vi "move folder contents up one hierarchy level.vi"(10 "error in":errorcluster, 11 "file":path) -> (2 "error out":errorcluster)   [LabVIEW 2014]
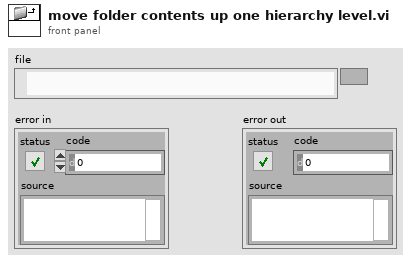
[diagram p1: front panel]
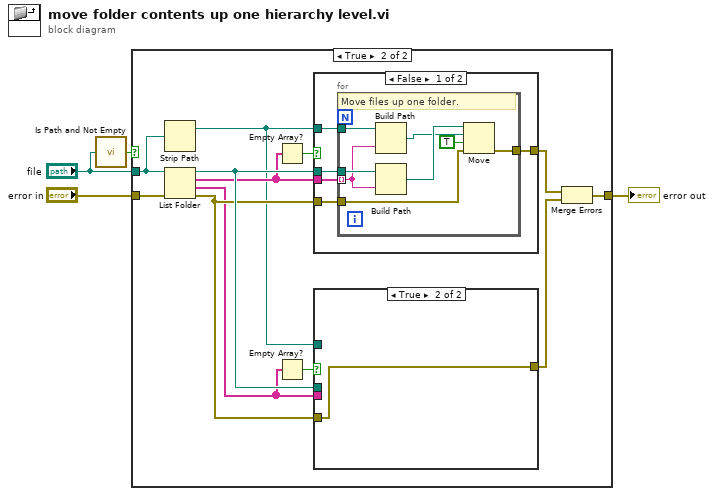
[diagram p0: block diagram]
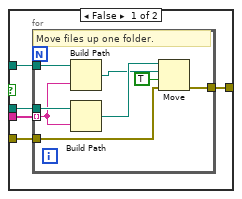
[diagram p3: hidden frame]
diagram:
  n1 = call <vilib>:"Is Path and Not Empty.vi"("path"="file") -> ("Is Path and Not Empty?"=w1:bool)  [unwired: 4 in]
  n2 = case shown="True" w1 {
    tunnel: "error in" -> [w5 w17]
    tunnel: [w5 w13] -> w3
    tunnel: "file" -> [_ w12]
    frame False {
    }
    frame True {
      n3 = Strip Path(path=w12) -> (stripped path=w10:path)  [unwired: 1 out]
      n4 = List Folder(path=w12, error in=w17) -> (path out=w16:path, filenames=w11:string[], folder names=w7:string[], error out=w15:errorcluster)  [unwired: 2 in]
      n5 = Empty Array?(array=w11) -> (empty?=w9:bool)
      n6 = Empty Array?(array=w7) -> (empty?=w8:bool)
      n7 = case shown="False" w9 {
        tunnel: w11 -> [w36 _]
        tunnel: w16 -> [w35 _]
        tunnel: w10 -> [w34 _]
        tunnel: w15 -> [w33 w45]
        tunnel: [w32 w45] -> w14
        frame False {
          n8 = for {
            tunnel: w35 -> [w44]
            tunnel: w36 -> [w41] mode=indexing
            tunnel: w34 -> [w42]
            tunnel: w33 -> [w39]
            tunnel: [w38] -> w32
            # "Move files up one folder."
            n9 = Build Path(base path=w42, name or relative path=w41) -> (appended path=w40:path)
            n10 = Build Path(base path=w44, name or relative path=w41) -> (appended path=w43:path)
            n11 = Move(source path=w43, error in=w39, 9:TRUE ("overwrite (F)"), 10:w40) -> (error out=w38:errorcluster)  [unwired: 1 in, 2 out]
          }
        }
        frame True {
        }
      }
      n12 = case shown="True" w8 {
        tunnel: w7 -> [w22 _]
        tunnel: w16 -> [w21 _]
        tunnel: w10 -> [w20 _]
        tunnel: w15 -> [w19 w31]
        tunnel: [w18 w31] -> w6
        frame False {
          n13 = for {
            tunnel: w21 -> [w30]
            tunnel: w22 -> [w27] mode=indexing
            tunnel: w20 -> [w28]
            tunnel: w19 -> [w25]
            tunnel: [w24] -> w18
            # "Move files up one folder."
            n14 = Build Path(base path=w28, name or relative path=w27) -> (appended path=w26:path)
            n15 = Build Path(base path=w30, name or relative path=w27) -> (appended path=w29:path)
            n16 = Move(source path=w29, error in=w25, 9:TRUE ("overwrite (F)"), 10:w26) -> (error out=w24:errorcluster)  [unwired: 1 in, 2 out]
          }
        }
        frame True {
        }
      }
      n17 = Merge Errors(w14, w6) -> (w13:errorcluster)
    }
  }
  "error out" <- w3
